vi "Free Part Num String.vi"(8 "error in (no error)":errorcluster caption="错误输入（无错误）", 11 "strPartNum":string) -> (0 "error out":errorcluster caption="错误输出", 3 "strPartNum out":string)   [LabVIEW 2017, in "smncsftmt.lvlib"]
doc: "__declspec(dllexport) void FreePartNumString(char* strPartNum);"
uses:
  smncsftmt.lvlib
  smncsftmt.dll
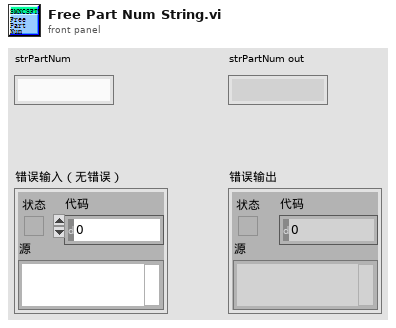
[diagram p1: front panel]
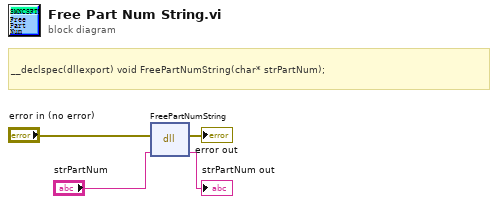
[diagram p0: block diagram]
diagram:
  # "__declspec(dllexport) void FreePartNumString(char* strPartNum);"
  n1 = dll-call lib="PTH2oabs CUsersaDesktop\nLABVIEW范例National InstrumentsLabVIEW 2017user.lib\tsmncsftmtsmncsftmt.*" fn="FreePartNumString"(error in="error in (no error)", "strPartNum"="strPartNum") -> (error out=→"error out":errorcluster, "strPartNum"=→"strPartNum out":string)  [unwired: 3 in, 1 out]
